vi "catch me if u can.vi"() -> ()   [LabVIEW 2018]
uses:
  <vilib>/Utility/miscctls.llb/LVPositionTypeDef.ctl
panel:
  out "Position":T1
  in  "NAHH BRO":bool
  in  "YES":bool
  # "Unnal Mudiyaath thambi"
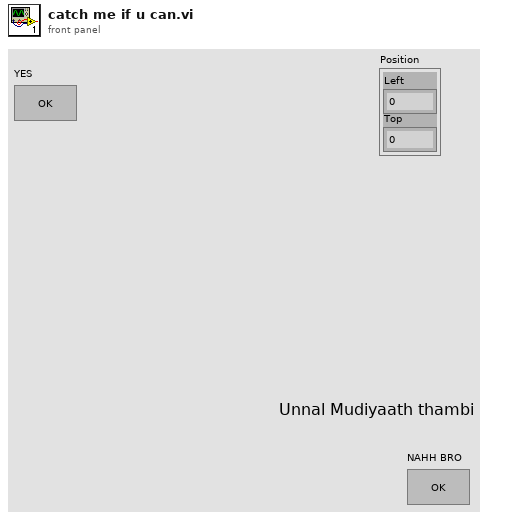
[diagram p1: front panel]
types:
  T1 = typedef "LVPositionTypeDef.ctl" = cluster{"Left":i32, "Top":i32}
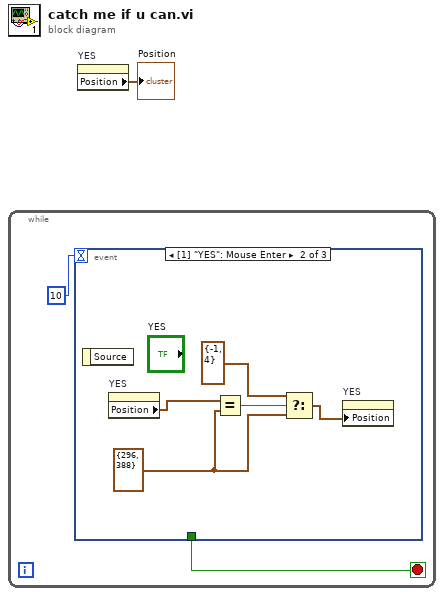
[diagram p0: block diagram]
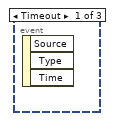
[diagram p2: hidden frame]
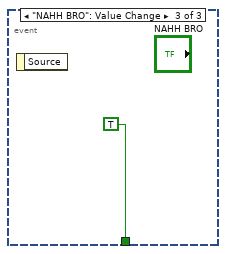
[diagram p3: hidden frame]
diagram:
  n1 = while {
    stop <- w2 stop-if-true
    n2 = event shown="[1] \"YES\": Mouse Enter" {
      selector: _ -> [_ _ _]
      dyn-events: _ -> [_ _ _]
      timeout: 10 -> [_ _ _]
      tunnel: [_ _ TRUE] -> w2
      event Timeout {
        n3 = event-data() -> ()  [unwired: 1 in, 3 out]
      }
      event "YES": Mouse Enter {
        w5 = T1 {"Left"=296, "Top"=388} ("Position")
        n4 = event-data() -> ()  [unwired: 1 in, 1 out]
        n5 = property on="YES" class="Bool"() -> ("Position"=w8:T1)  [unwired: 2 in, 2 out]
        n6 = Equal?(x=w8, y=w5) -> (x = y?=w7:bool)
        n7 = Select(t=T1 {"Left"=-1, "Top"=4} ("Position"), s=w7, f=w5) -> (s? t:f=w4:T1)
        n8 = property on="YES" class="Bool"("Position"=w4) -> ()  [unwired: 2 in, 2 out]
      }
      event "NAHH BRO": Value Change {
        n9 = event-data() -> ()  [unwired: 1 in, 1 out]
      }
    }
  }
  n10 = property on="YES" class="Bool"() -> ("Position"=→"Position":T1)  [unwired: 2 in, 2 out]
